vi "csb encode pcap to ws.vi"(0 "in":u8[](array[numeric]), 1 "out":u8[](array[numeric])=array[4097 elements], 5 "in_len":i32, 7 "options":i32, 9 "mask":u32, 11 "error in (no error)":errorcluster, 12 "out_cap":i32) -> (3 "out out":u8[](array[numeric]), 4 "n_packets":i32, 6 "n_rejected":i32, 8 "consumed":i32, 10 "function return":i32, 15 "error out":errorcluster)   [LabVIEW 2021, in "CANsub_Codec.lvlib"]
doc: "int32_t csb_encode_pcap_to_ws(const uint8_t *in, int32_t in_len, int32_t options, uint32_t mask,\n uint8_t *out, int32_t out_cap,\n int32_t *n_packets, int32_t *n_rejected, int32_t *consumed);"
uses:
  CANsub_Codec.lvlib
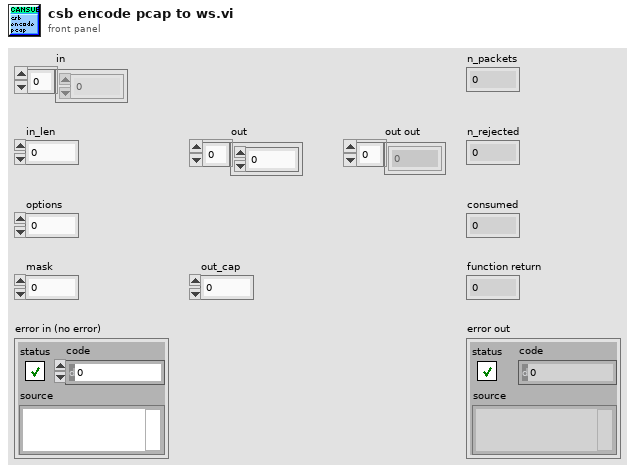
[diagram p1: front panel]
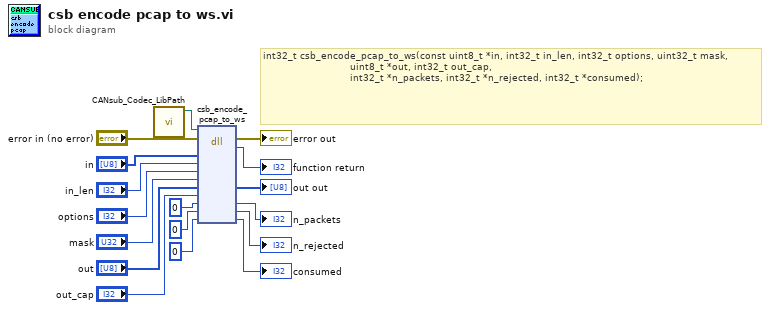
[diagram p0: block diagram]
diagram:
  # "int32_t csb_encode_pcap_to_ws(const uint8_t *in, int32_t in_len, int32_t options, uint32_t mask,\n                             uint8_t *out, int32_t out_cap,\n                             int32_t *n_packets, int32_t *n_rejected, int32_t *consumed);"
  n1 = call "CANsub_Codec_LibPath.vi"() -> ("Path"=w1:path)  [unwired: 11 in]
  n2 = dll-call lib="libcansub_codec.*" fn="csb_encode_pcap_to_ws"(path in=w1, error in="error in (no error)", "in"="in", "in_len"="in_len", "options"="options", "mask"="mask", "out"="out", "out_cap"="out_cap", "n_packets"=0, "n_rejected"=0, "consumed"=0) -> (error out=→"error out":errorcluster, "return type"=→"function return":i32, "out"=→"out out":u8[], "n_packets"=→"n_packets":i32, "n_rejected"=→"n_rejected":i32, "consumed"=→"consumed":i32)  [unwired: 6 in, 1 out]
